vi "RDB Parse.vi"(8 "error in (no error)":errorcluster, 10 "RDB Message":string, 11 "Settings":T1={"UDP Receiver"=refnum, "UDP Sender"=refnum, "Valid Packet"=FALSE, "TCP"=refnum, "Network Settings"={"IP adress"="127.0.0.1", "RDB"={"Protocol"=enum."UDP", "Tx Port"=48270, "Rx Port"=10, "Buffer Size"=204800, "Timeout"=10}, "SCP"={"Protocol"=enum."TCP", "Tx Port"=48191, "Rx Port"=48191, "Buffer Size"=204800, "Timeout"=10}}, "vclient"=path "", "paeseHandle"=0, "builderHandle"=0}) -> (0 "error out":errorcluster, 1 "simFrame":dbl, 2 "simTime":dbl, 3 "Settings":T1={"UDP Receiver"=refnum, "UDP Sender"=refnum, "Valid Packet"=FALSE, "TCP"=refnum, "Network Settings"={"IP adress"="127.0.0.1", "RDB"={"Protocol"=enum."UDP", "Tx Port"=48270, "Rx Port"=10, "Buffer Size"=204800, "Timeout"=10}, "SCP"={"Protocol"=enum."TCP", "Tx Port"=48191, "Rx Port"=48191, "Buffer Size"=204800, "Timeout"=10}}, "vclient"=path "", "paeseHandle"=0, "builderHandle"=0})   [LabVIEW 2023, in "RDB.lvlib"]
uses:
  RDB.lvlib
  Engine/Type/Settings.ctl
  Shared/Network Settings.ctl
  Shared/Protocol.ctl
  Engine/Vires VTD Engine.lvlib
  Shared/Vires VTD Shared.lvlib
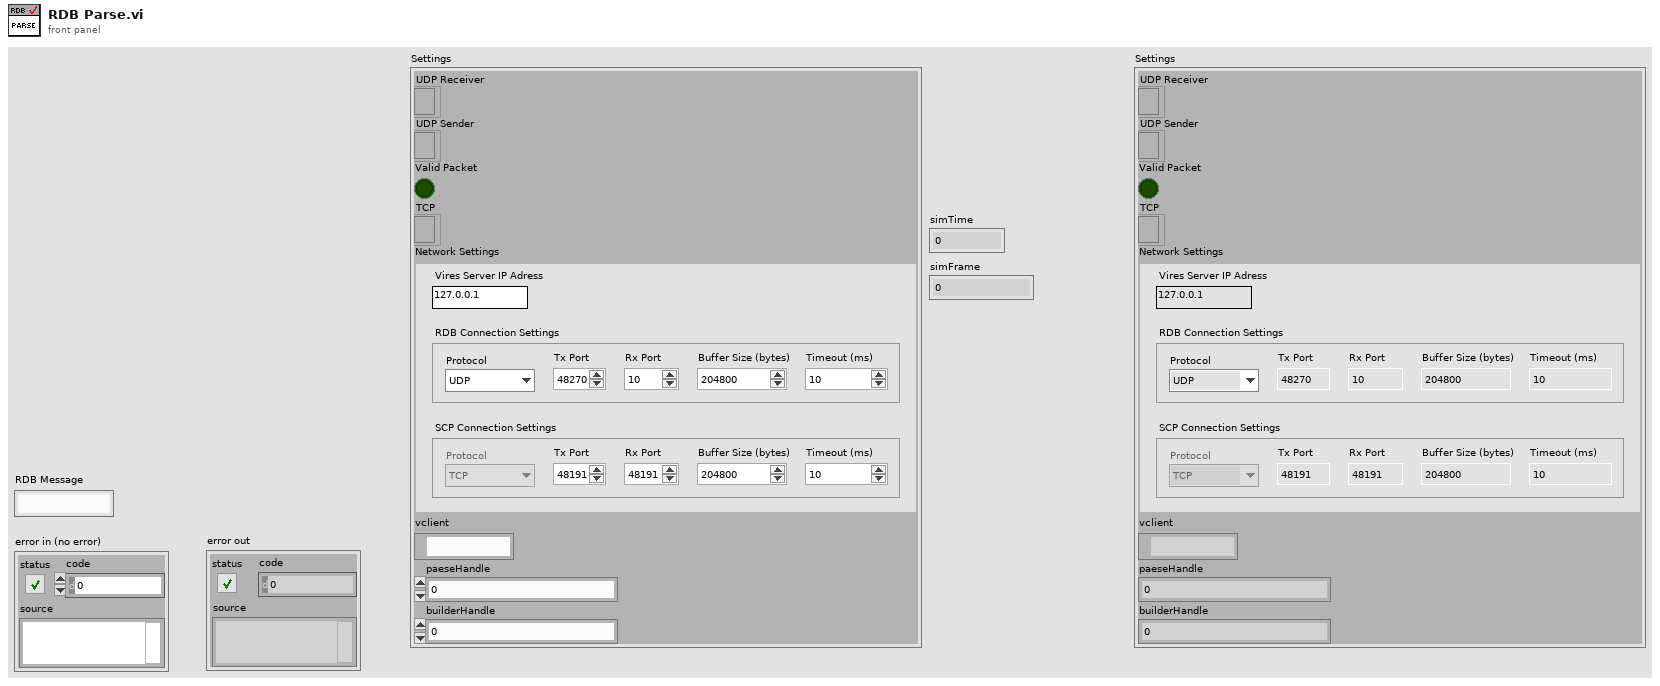
[diagram p1: front panel]
types:
  T1 = typedef "Vires VTD Engine.lvlib/Settings.ctl" = cluster{"UDP Receiver":refnum<k16>, "UDP Sender":refnum<k16>, "Valid Packet":bool, "TCP":refnum<k5>, "Network Settings":T2, "vclient":path, "paeseHandle":u64, "builderHandle":u64}
  T2 = typedef "Vires VTD Shared.lvlib/Network Settings.ctl" = cluster{"IP adress":string, "RDB":cluster{"Protocol":T3, "Tx Port":u16, "Rx Port":u16, "Buffer Size":i32, "Timeout":u16}, "SCP":cluster{"Protocol":T3, "Tx Port":u16, "Rx Port":u16, "Buffer Size":i32, "Timeout":u16}}
  T3 = typedef "Vires VTD Shared.lvlib/Protocol.ctl" = enum16{"UDP", "TCP"}
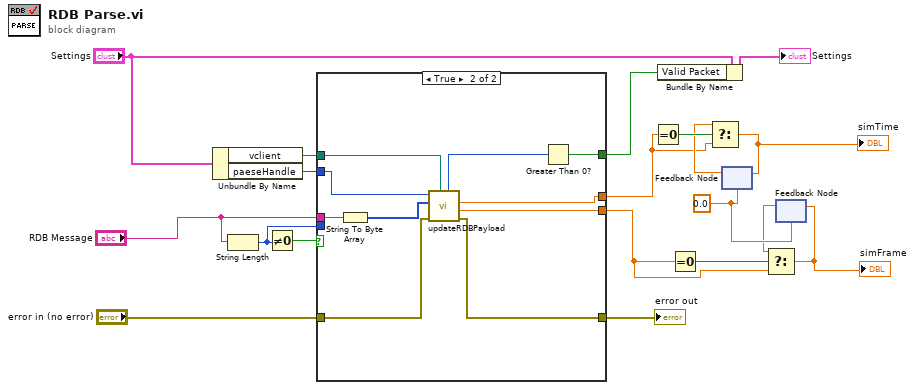
[diagram p0: block diagram]
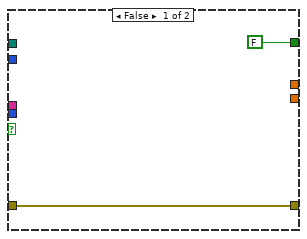
[diagram p2: hidden frame]
diagram:
  w9 = 0.0
  n1 = Unbundle By Name("Settings") -> ("vclient"=w12:path, "paeseHandle"=w10:u64)
  n2 = String Length(string="RDB Message") -> (length=w13:i32)
  n3 = Not Equal To 0?(x=w13) -> (x != 0?=w16:bool)
  n4 = case shown="True" w16 {
    tunnel: "error in (no error)" -> [w21 w25]
    tunnel: [w21 w24] -> w18
    tunnel: "RDB Message" -> [_ w27]
    tunnel: [FALSE w31] -> w14
    tunnel: w13 -> [_ _]
    tunnel: w12 -> [_ w30]
    tunnel: w10 -> [_ w29]
    tunnel: [_ w23] -> w2
    tunnel: [_ w22] -> w4
    frame False {
    }
    frame True {
      n5 = String To Byte Array(string=w27) -> (unsigned byte array=w26:u8[])
      n6 = call "updateRDBPayload.vi"("path in"=w30, "error in (no error)"=w25, "payload"=w26, "paeseHandle in"=w29) -> ("error out"=w24:errorcluster, "simFrame"=w23:dbl, "simTime"=w22:dbl, "isComplete"=w28:u8)  [unwired: 3 in, 1 out]
      n7 = Greater Than 0?(x=w28) -> (x > 0?=w31:bool)
    }
  }
  "error out" <- w18
  n8 = Equal To 0?(x=w4) -> (x = 0?=w8:bool)
  n9 = Bundle By Name(cluster="Settings", "Valid Packet"=w14) -> (→"Settings":T1)
  n10 = Equal To 0?(x=w2) -> (x = 0?=w6:bool)
  n11 = feedback #1(w9) -> (w7:dbl)
  n12 = Select(t=w7, s=w8, f=w4) -> (s? t:f=w5:dbl)
  "simTime" <- w5
  n13 = feedback-in #1(w5) -> ()
  n14 = feedback #2(w9) -> (w3:dbl)
  n15 = Select(t=w3, s=w6, f=w2) -> (s? t:f=w1:dbl)
  "simFrame" <- w1
  n16 = feedback-in #2(w1) -> ()
